vi "DAQ Cal Info.vi"() -> (3 "DevTemp":dbl)   [LabVIEW 2013]
uses:
  <resource>/objmgr/daqmx.rc
panel:
  out "ExtCal.RecommendedInterval":u32
  out "SelfCal.LastDate/Time":timestamp
  out "SelfCal.Supported":bool
  out "SelfCal.LastTemp":dbl
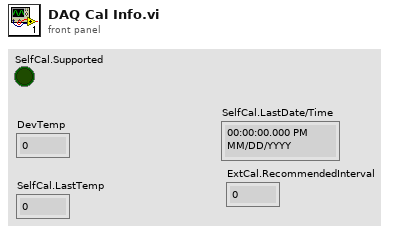
[diagram p1: front panel]
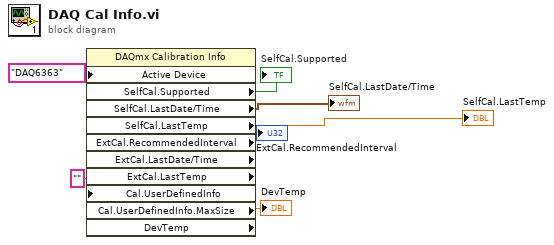
[diagram p0: block diagram]
diagram:
  n1 = property class="DAQmx Calibration Info" props=["Active Device", "SelfCal.Supported", "SelfCal.LastDate/Time", "SelfCal.LastTemp", "ExtCal.RecommendedInterval", "ExtCal.LastDate/Time", "ExtCal.LastTemp", "Cal.UserDefinedInfo", "Cal.UserDefinedInfo.MaxSize", "DevTemp"]("Active Device"=tag "DAQ6363" ("ActiveDev"), "Cal.UserDefinedInfo"="") -> ("SelfCal.Supported"=→"SelfCal.Supported":bool, "SelfCal.LastDate/Time"=→"SelfCal.LastDate/Time":timestamp, "SelfCal.LastTemp"=→"SelfCal.LastTemp":dbl, "ExtCal.RecommendedInterval"=→"ExtCal.RecommendedInterval":u32, "DevTemp"=→"DevTemp":dbl)  [unwired: 2 in, 5 out]
